vi "查找DAQ.vi"(8 "允许仿真":bool, 10 "表达式":string) -> (0 "error out":errorcluster caption="错误输出", 2 "DAQmx设备名":tag)   [LabVIEW 2025]
uses:
  <vilib>/regexp/Match Regular Expression.xnode
  <resource>/objmgr/daqmx.rc
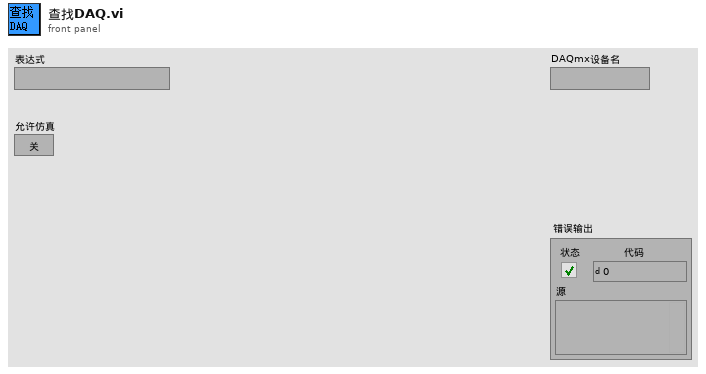
[diagram p1: front panel]
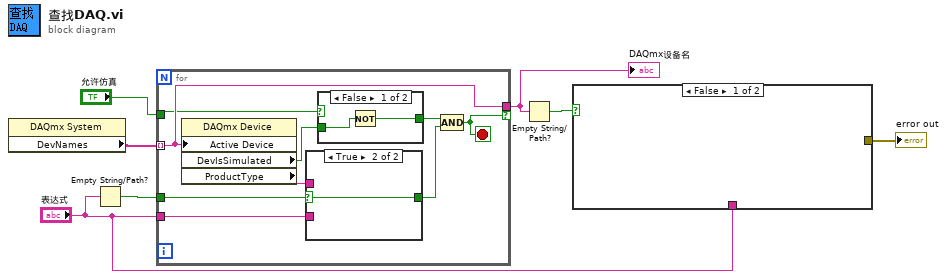
[diagram p0: block diagram]
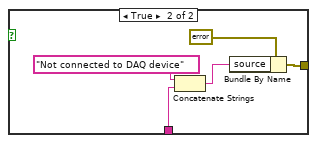
[diagram p2: hidden frame]
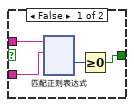
[diagram p4: hidden frame]
diagram:
  n1 = property class="DAQmx System"() -> ("DevNames"=w7:tag[])  [unwired: 2 in, 2 out]
  n2 = Empty String/Path?(string/path="表达式") -> (empty?=w2:bool)
  n3 = for {
    tunnel: w7 -> [w15] mode=indexing
    tunnel: "表达式" -> [w12]
    tunnel: [w15] -> w6 if=w14
    tunnel: "允许仿真" -> [w10]
    tunnel: w2 -> [w11]
    stop <- w14 stop-if-true
    n4 = property class="DAQmx Device"("Active Device"=w15) -> ("DevIsSimulated"=w9:bool, "ProductType"=w13:string)  [unwired: 2 in, 2 out]
    n5 = case shown="True" w11 {
      selector: w11 -> [_ w141]
      tunnel: [w23 w141] -> w16
      tunnel: w13 -> [w22 _]
      tunnel: w12 -> [w20 _]
      frame False {
        n6 = xnode "匹配正则表达式"("input string"=w22, "regular expression"=w20) -> ("offset past match"=w21:i32)  [unwired: 4 in, 4 out]
        n7 = Greater Or Equal To 0?(x=w21) -> (x >= 0?=w23:bool)
      }
      frame True {
      }
    }
    n8 = case shown="False" w10 {
      tunnel: w9 -> [w18 w19]
      tunnel: [w17 w19] -> w8
      frame False {
        n9 = Not(x=w18) -> (.not. x?=w17:bool)
      }
      frame True {
      }
    }
    n10 = Compound Arithmetic op=AND(w8, w16) -> (w14:bool)
  }
  "DAQmx设备名" <- w6
  n11 = Empty String/Path?(string/path=w6) -> (empty?=w5:bool)
  n12 = case shown="False" w5 {
    tunnel: [_ w145] -> w4
    tunnel: "表达式" -> [_ w142]
    frame False {
    }
    frame True {
      n13 = Concatenate Strings("Not connected to DAQ device", w142) -> (w143:string)
      n14 = Bundle By Name(cluster=errorcluster {"status"=TRUE, "code"=0, "source"=""} ("错误常量"), "source"=w143) -> (w145:errorcluster)
    }
  }
  "error out" <- w4
